vi "niGPS Direct Streaming.vi"() -> ()   [LabVIEW 2026]
doc: "This example shows how to simulate GPS signals using a real receiver location. This example also demonstrates the generation of GPS data without storing it into an intermediate binary file. The signal simulation is done based on the user input for Almanac File, Ephemeris File, Initial GPS Time of Week, Number of Frames, Receiver Location Format and Receiver Location and Receiver Velocity. The Data Creation Mode has been chosen to be Automatic. This guarantees a position fix in almost all the cases provided that the receiver location is valid and the sufficient satellites have passed the checks to be selected in simulation. \n\n\nSample ECEF values in the order of X,Y,Z in meters for different locations:\n\n\nBangalore (India) : 1.33678E+6, 6.07161E+6, 1.42381E+6 \nAustin (USA): -742817, -5.46326E+6, 3.19603E+6\nFlorence (Italy) : 4.52486E+6, 900051, 4.38947E+6 \nBrussels (Belgium) : 4.02493E+6, 304989, 4.92191E+6 \nVimercate (Italy) : 4.40941E+6, 727340, 4.53568E+6\n\nYou can find the coordinates of places easily on the web. One example is : Visit:http://www.fallingrain.com/world/"
uses:
  <vilib>/addons/Modulation/Analog/controls/Complex Data Waveform.ctl
  <vilib>/addons/Modulation/Analog/support/Validators/mod_Fractional Resample Validate.vi
  <vilib>/addons/Modulation/Analog/support/Validators/mod_Check Flush State.vi
  <vilib>/addons/Modulation/Analog/support/mod_FractionalResampler.vi
  <vilib>/addons/Modulation/Analog/support/mod_Integer Rate Interpolation.vi
  <vilib>/addons/Modulation/Analog/support/mod_Set Error Source.vi
  <vilib>/addons/Modulation/Analog/support/Validators/mod_Validate Complex Waveform.vi
  <vilib>/addons/Modulation/Analog/support/mod_PerformResampling.vi
  <vilib>/addons/Modulation/Analog/support/Validators/mod_WFErrorHandler.vi
  <instrlib>/niUSRP/niUSRP Write Tx Data (CDB Cluster).vi
  <vilib>/Utility/error.llb/Error Cluster From Error Code.vi
  <vilib>/addons/Modulation/Analog/support/mod_Resampling Factors.vi
  <vilib>/addons/Modulation/Analog/support/mod_ResamplingFilter.vi
  <vilib>/addons/Modulation/Analog/support/mod_Generate Integer Interpolation Filter.vi
  <resource>/objmgr/niGPSAttribs.rc
  <vilib>/addons/Modulation/niAMT.lvlib
panel:
  out "Waveform Graph":cluster{"t0":dbl, "dt":dbl, "Y":dbl[]}(graph)
  in  "Reference Frequency Source":string(combo)="GPS"
  in  "Stop Generation":bool
  in  "Generate GPS":bool
  in  "Freq Offset, Hz":dbl=4000000.0 format="%^.2e"
  out "coerced carrier":dbl=1575420000.0099506 format="%#_6p"
  out "coerced IQ rate":dbl=2000000.0 format="%#_6p"
  in  "device names":refnum<k15>="192.168.10.2"
  in  "IQ rate (S/s)":dbl=2000000.0 format="%#_6p"
  in  "carrier frequency":dbl=1575420000.0 format="%#_6p"
  in  "Gain":dbl format="%.2f"
  out "Consumer End":bool
  out "Producer End":bool
  out "Queue":i32(slide)=100 scale=0.0..100.0
  in  "Waveform Scaling Factor":dbl=0.5
  in  "Max Relative Power Level (dB)":dbl=10.0
  in  "Optimal Satellite Update Interval":dbl=30.0
  in  "Maximum Number of \nOptimal Satellites":i32=8
  out "Satellites Selected":string="2,5,6,7,10,12,24,30"
  out "Generation State":T1(ring)=enum."Generating Waveform"
  in  "Initial GPS Time of Week":u32=345600
  in  "Reference Power Level (dBm)":dbl=-50.0
  out "Number of Bits Created":i32(slide)=916 scale=0.0..37500.0
  out "Current GPS Time of Week":dbl=345782.82 format="%.4f"
  in  "Receiver Location":enum32{"ECEF", "LLA "}(tab)=enum."LLA "
  in  "Z":dbl=3196033.0 format="%#_f"
  in  "Y":dbl=-5463257.0 format="%#_f"
  in  "X":dbl=-742817.0 format="%#_f"
  in  "LLA":enum32{"Latitude", "Longitude", "Altitude"}(tab)
  in  "Lat.Direction":i32(ring) items=["N", "S"]
  in  "Lat.Seconds":dbl=26.3754
  in  "Lat.Minutes":dbl=50.0
  in  "Lat.Degrees":dbl=38.0
  in  "Long.Direction":i32(ring)=1 items=["E", "W"]
  in  "Long.Seconds":dbl=38.7132
  in  "Long.Minutes":dbl=2.0
  in  "Long.Degrees":dbl=105.0
  in  "Altitude":dbl=4302.0
  in  "Number of Frames":i32=25
  in  "Receiver Location Format":i32(ring)=1 items=["ECEF", "LLA"]
  in  "Ephemeris File Path":path=path "C:/Program Files (x86)/National Instruments/GPS/Ephemeris files/brdc3190.07n"
  in  "Almanac File Path":path=path "C:/Program Files (x86)/National Instruments/GPS/Almanac files/319.al3"
  out "Error Out":errorcluster
  # "NI-USRP CONFIG"
  # "GPS SETTINGS"
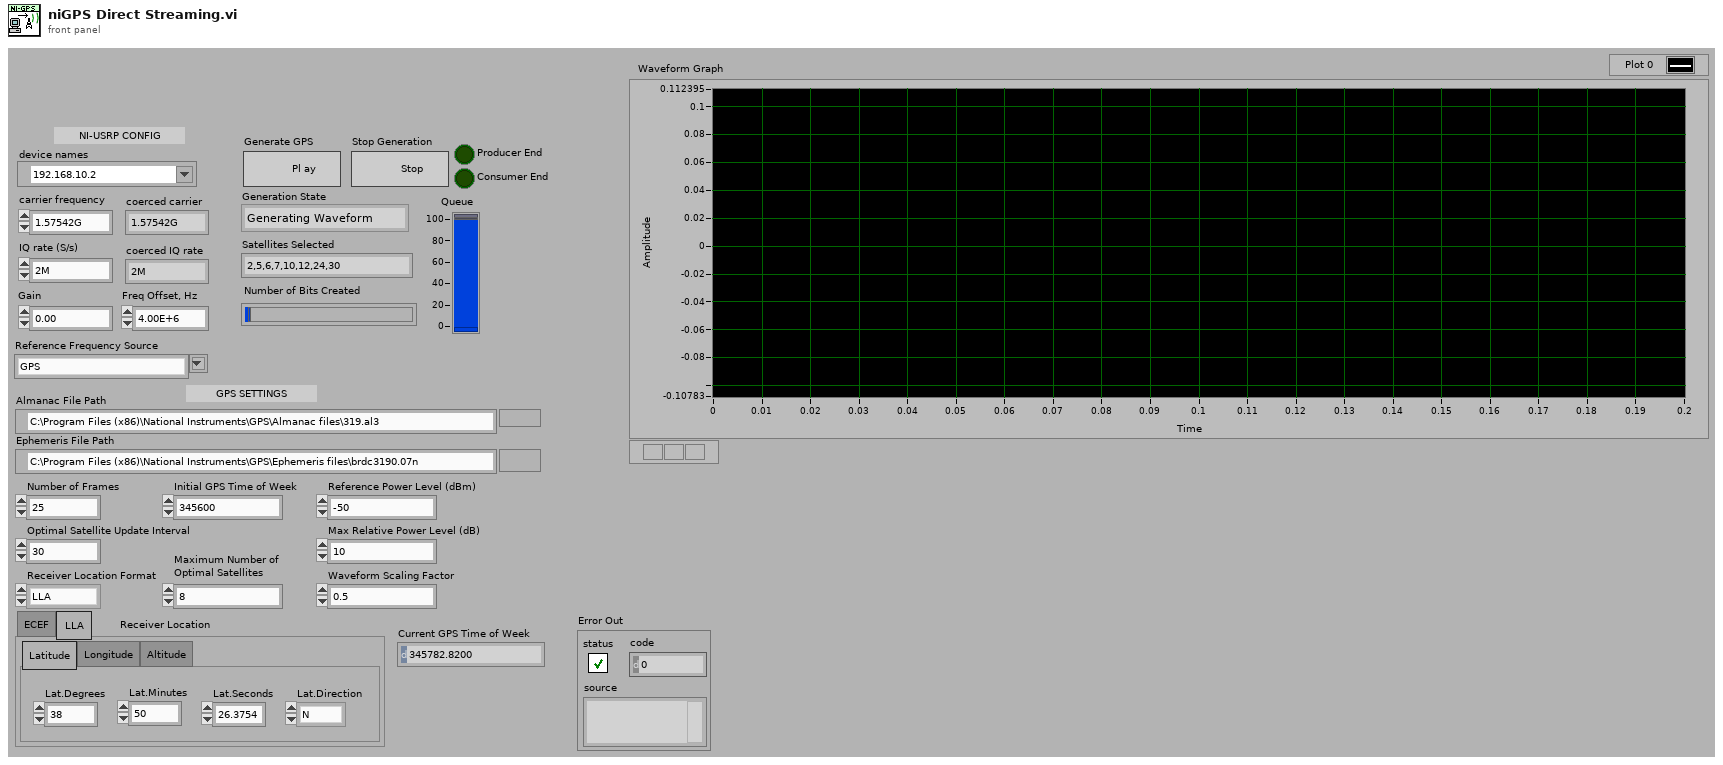
[diagram p1: front panel]
types:
  T1 = enum16{"Not Generating", "Buffering Waveform", "Generating Waveform", "Finishing Generation"}
  T2 = typedef "niAMT.lvlib/Complex Data Waveform.ctl" = cluster{"t0":dbl, "dt":dbl, "Y":cdb[]}
  T3 = typedef "gpsv1_refnum.ctl" = refnum<k20>
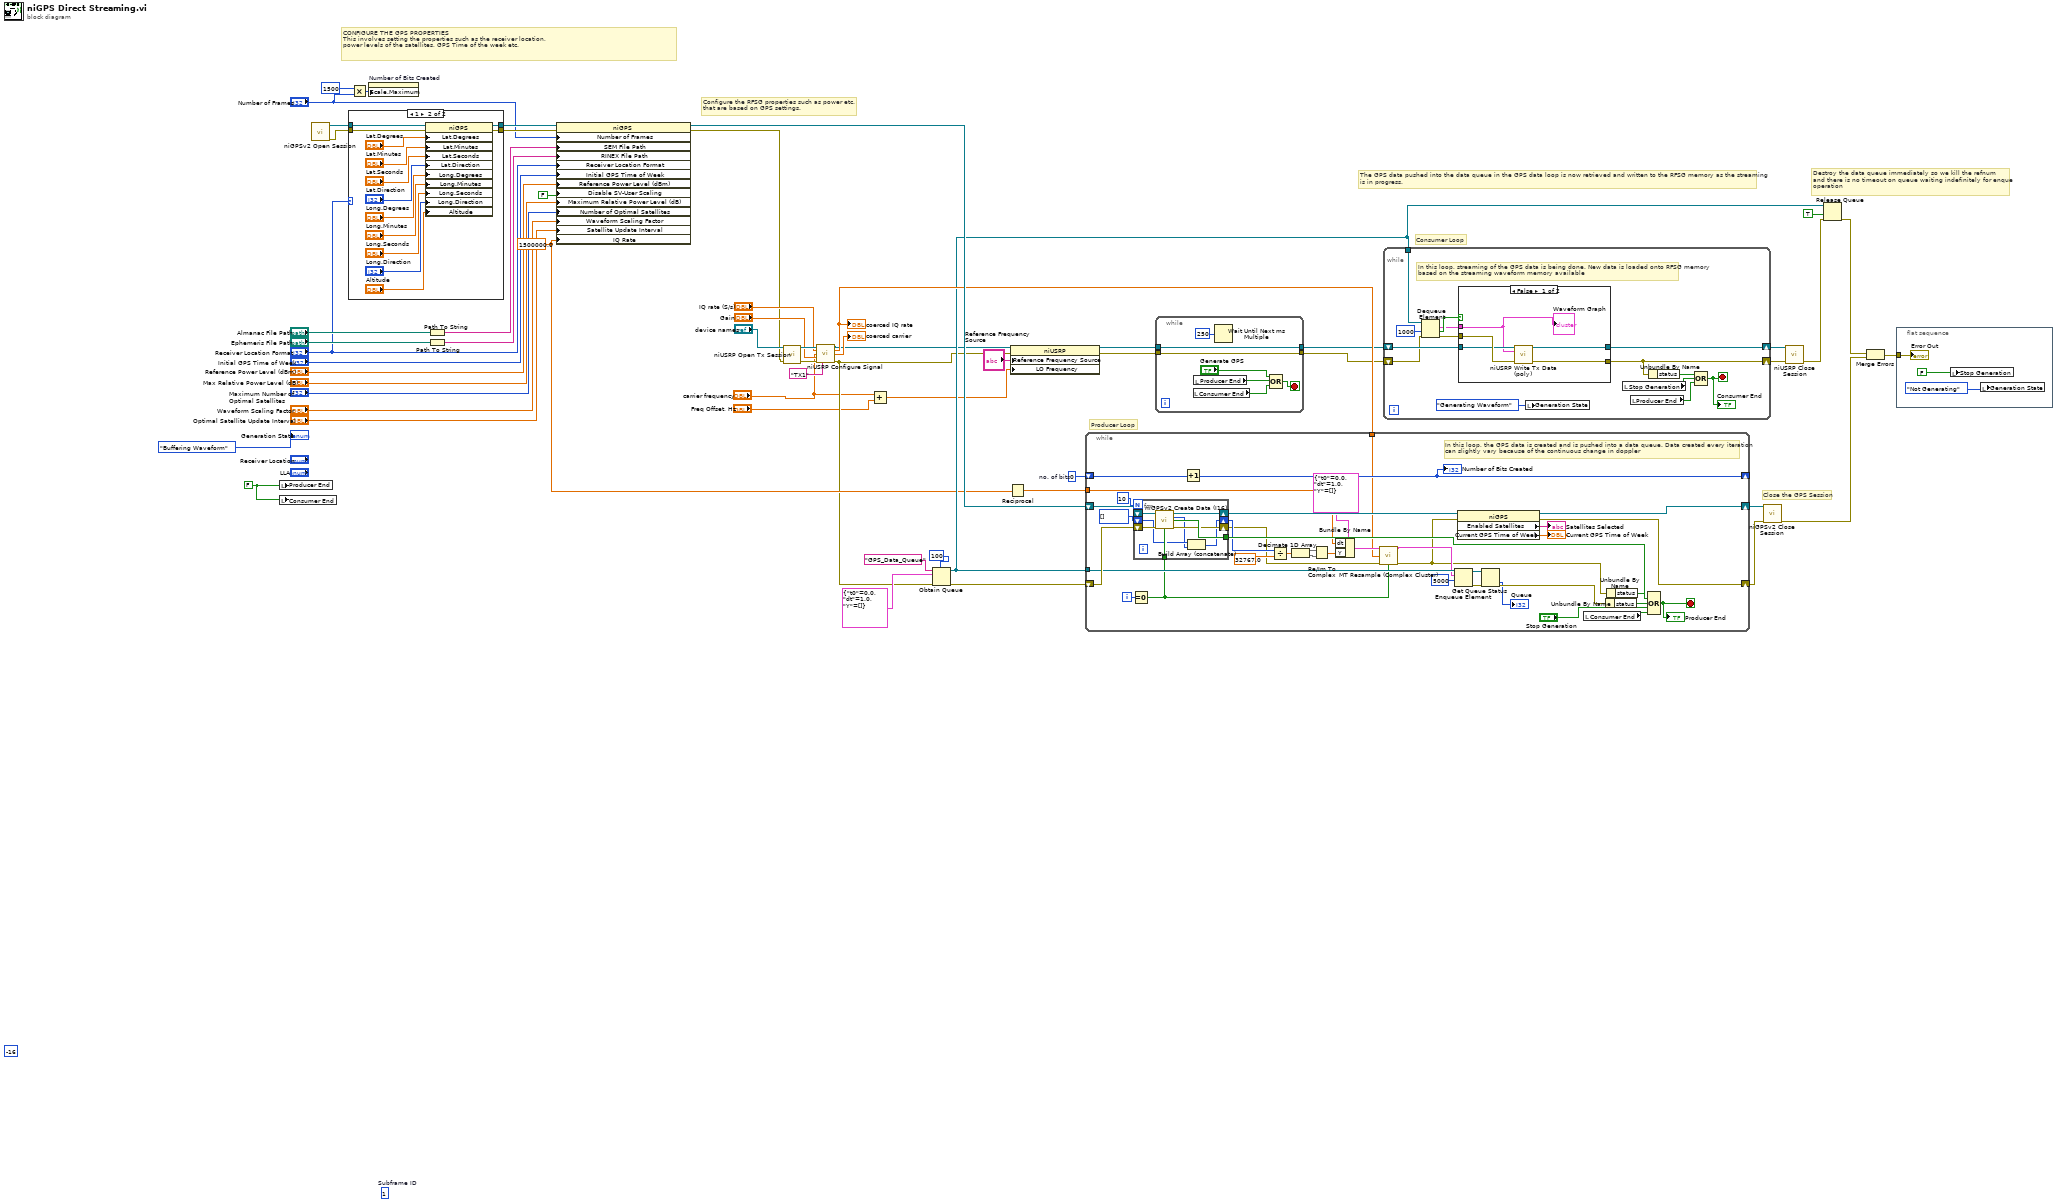
[diagram p0: block diagram]
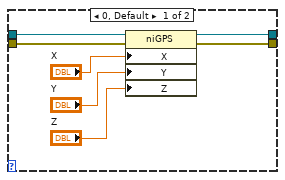
[diagram p3: hidden frame]
diagram:
  w14 = 1500000.0 ("IQ Rate")
  w31 = FALSE ("Producer End")
  w38 = 0  # no. of bits
  (unwired) i16 -16 ("n")
  (unwired) i8 1  # Subframe ID
  # "Producer Loop"
  # "Consumer Loop"
  # "The GPS data pushed into the data queue in the GPS data loop is now retrieved and written to the RFSG memory as the streaming \nis in progress."
  # "Configure the RFSG properties such as power etc. \nthat are based on GPS settings."
  # "Close the GPS Session"
  # "Destroy the data queue immediately so we kill the refnum \nand there is no timeout on queue waiting indefinitely for enque \noperation"
  # "CONFIGURE THE GPS PROPERTIES \nThis involves setting the properties such as the receiver location, \npower levels of the satellites, GPS Time of the week etc."
  n1 = local write "Producer End"(w31) -> ()
  n2 = local write "Consumer End"(w31) -> ()
  n3 = call <vilib>:"niGPSv2 Open Session.vi"() -> ("nigps session out"=w54:T3, "error out"=w34:errorcluster)  [unwired: 14 in]
  n4 = case shown="1" "Receiver Location Format" {
    tunnel: w54 -> [w65 w77]
    tunnel: w34 -> [w63 w76]
    tunnel: [w64 w78] -> w45
    tunnel: [w62 w75] -> w53
    frame 0, Default {
      n5 = property class="niGPS"(reference=w65, error in=w63, "X"="X", "Y"="Y", "Z"="Z") -> (reference out=w64:T3, error out=w62:errorcluster)
    }
    frame 1 {
      n6 = property class="niGPS"(reference=w77, error in=w76, "Lat.Degrees"="Lat.Degrees", "Lat.Minutes"="Lat.Minutes", "Lat.Seconds"="Lat.Seconds", "Lat.Direction"="Lat.Direction", "Long.Degrees"="Long.Degrees", "Long.Minutes"="Long.Minutes", "Long.Seconds"="Long.Seconds", "Long.Direction"="Long.Direction", "Altitude"="Altitude") -> (reference out=w78:T3, error out=w75:errorcluster)
    }
  }
  n7 = Multiply(x=1500, y="Number of Frames") -> (x*y=w51:i32)
  n8 = property on="Number of Bits Created" class="Slide (strict)"("Scale.Maximum"=w51) -> ()  [unwired: 2 in, 2 out]
  n9 = Path To String(path="Almanac File Path") -> (string=w55:string)
  n10 = Path To String(path="Ephemeris File Path") -> (string=w58:string)
  n11 = property class="niGPS"(reference=w45, error in=w53, "Number of Frames"="Number of Frames", "SEM File Path"=w55, "RINEX File Path"=w58, "Receiver Location Format"="Receiver Location Format", "Initial GPS Time of Week"="Initial GPS Time of Week", "Reference Power Level (dBm)"="Reference Power Level (dBm)", "Disable SV-User Scaling"=FALSE, "Maximum Relative Power Level (dB)"="Max Relative Power Level (dB)", "Number of Optimal Satellites"="Maximum Number of \nOptimal Satellites", "Waveform Scaling Factor"="Waveform Scaling Factor", "Satellite Update Interval"="Optimal Satellite Update Interval", "IQ Rate"=w14) -> (reference out=w30:T3, error out=w10:errorcluster)
  n12 = call <instrlib>:"niUSRP Open Tx Session.vi"("device names"="device names", "error in (no error)"=w10) -> ("session handle out"=w29:refnum<k15>, "error out"=w9:errorcluster)  [unwired: 12 in]
  n13 = call <instrlib>:"niUSRP Configure Signal.vi"("session handle"=w29, "IQ rate"="IQ rate (S/s)", "carrier frequency"="carrier frequency", "gain"="Gain", "error in (no error)"=w9, "active antenna"="TX1") -> ("session handle out"=w13:refnum<k15>, "coerced IQ rate"=w17:dbl, "coerced carrier frequency"=→"coerced carrier":dbl, "error out"=w11:errorcluster)  [unwired: 5 in, 1 out]
  "coerced IQ rate" <- w17
  n14 = Add(x="carrier frequency", y="Freq Offset, Hz") -> (x+y=w1:dbl)
  n15 = Obtain Queue(max queue size (-1, unlimited)=100, name (unnamed)="GPS_Data_Queue", element data type=T2 {"t0"=0.0, "dt"=1.0, "Y"=[]} ("input complex waveform"), error in (no error)=w11) -> (queue out=w16:refnum<queue>, error out=w36:errorcluster)  [unwired: 1 in, 1 out]
  n16 = Reciprocal(x=w14) -> (1/x=w19:dbl)
  n17 = property class="niUSRP"(reference=w13, error in=w11, "Reference Frequency Source"="Reference Frequency Source", "LO Frequency"=w1) -> (reference out=w8:refnum<k15>, error out=w7:errorcluster)
  n18 = while {
    shift-right: [w110] -> w32
    shift-left: w36 -> [w115]
    shift-right: [w111] -> w39
    shift-left: w30 -> [w116]
    shift-right: [w105] -> _
    shift-left: w38 -> [w106]
    tunnel: w19 -> [w84]
    tunnel: w17 -> [w90]
    tunnel: w16 -> [w86]
    i -> [w114]
    stop <- w85 stop-if-true
    # "In this loop, the GPS data is created and is pushed into a data queue. Data created every iteration\ncan slightly vary because of the continuous change in doppler"
    n19 = Equal To 0?(x=w114) -> (x = 0?=w82:bool)
    n20 = for {
      N: 10 -> [_]
      tunnel: w82 -> [w123]
      tunnel: [w121] -> w109
      shift-right: [w122] -> w112
      shift-left: w116 -> [w125]
      shift-right: [w117] -> w92
      shift-left: i16[] [] ("gps waveform") -> [w119]
      shift-right: [w120] -> w88
      shift-left: w115 -> [w124]
      n21 = call <vilib>:"niGPSv2 Create Data (I16).vi"("nigps session"=w125, "error in"=w124, "reset?"=w123) -> ("nigps session out"=w122:T3, "gps waveform"=w118:i16[], "done?"=w121:bool, "error out"=w120:errorcluster)  [unwired: 9 in]
      n22 = Build Array (concatenate)(w119, w118) -> (w117:i16[])
    }
    n23 = Increment(x=w106) -> (x+1=w105:i32)
    "Number of Bits Created" <- w105
    n24 = Divide(x=w92, y=32767.0 ("n")) -> (x/y=w89:dbl[])
    n25 = Decimate 1D Array(w89) -> (w93:dbl[], w94:dbl[])
    n26 = Re/Im To Complex(1:w94, 2:w93) -> (0:w83:cdb[])
    n27 = Bundle By Name(cluster=T2 {"t0"=0.0, "dt"=1.0, "Y"=[]} ("input complex waveform"), "dt"=w84, "Y"=w83) -> (w96:T2)
    n28 = call <vilib>:"MT Resample (Complex Cluster).vi"("input complex waveform"=w96, "desired sample rate (Hz)"=w90, "error in (no error)"=w88, "reset? (T)"=w82) -> ("output complex waveform"=w80:T2, "error out"=w79:errorcluster)  [unwired: 10 in]
    n29 = Enqueue Element(queue=w86, element=w80, timeout in ms (-1)=5000) -> (queue out=w104:refnum<queue>, error out=w103:errorcluster)  [unwired: 1 in, 1 out]
    n30 = property class="niGPS"(reference=w112, error in=w79) -> (reference out=w111:T3, error out=w110:errorcluster, "Enabled Satellites"=→"Satellites Selected":string, "Current GPS Time of Week"=→"Current GPS Time of Week":dbl)
    n31 = Get Queue Status(queue=w104, error in (no error)=w103) -> (error out=w102:errorcluster, # elements in queue=→"Queue":i32)  [unwired: 1 in, 6 out]
    n32 = local read "Consumer End"() -> (w101:bool)
    n33 = Unbundle By Name(w102) -> ("status"=w113:bool)
    n34 = Unbundle By Name(w79) -> ("status"=w99:bool)
    n35 = Compound Arithmetic op=OR(w99, w109, w113, "Stop Generation", w101) -> (w85:bool)
    "Producer End" <- w85
  }
  n36 = while {
    tunnel: w8 -> [w132]
    tunnel: w7 -> [w131]
    tunnel: [w132] -> w6
    tunnel: [w131] -> w5
    stop <- w129 stop-if-true
    n37 = local read "Consumer End"() -> (w126:bool)
    n38 = local read "Producer End"() -> (w127:bool)
    n39 = Wait Until Next ms Multiple(millisecond multiple=u32 250) -> ()  [unwired: 1 out]
    n40 = Compound Arithmetic op=OR("Generate GPS", w127, w126) -> (w129:bool)
  }
  n41 = while {
    shift-right: [w146] -> w23
    shift-left: w6 -> [w141]
    shift-right: [w145] -> w24
    shift-left: w5 -> [w136]
    tunnel: w16 -> [w134]
    stop <- w133 stop-if-true
    # "In this loop, streaming of the GPS data is being done. New data is loaded onto RFSG memory \nbased on the streaming waveform memory available"
    n42 = Dequeue Element(queue=w134, timeout in ms (-1)=1000, error in (no error)=w136) -> (element=w135:T2, timed out?=w138:bool, error out=w137:errorcluster)  [unwired: 1 out]
    n43 = case shown="False" w138 {
      tunnel: w141 -> [w148 w153]
      tunnel: [w150 w152] -> w145
      tunnel: [w151 w153] -> w146
      tunnel: w137 -> [w149 w152]
      tunnel: w135 -> [w147 _]
      frame False {
        n44 = call-poly <instrlib>:"niUSRP Write Tx Data (poly).vi"("session handle"=w148, "data"=w147, "error in (no error)"=w149) -> ("session handle out"=w151:refnum<k15>, "error out"=w150:errorcluster)  [unwired: 11 in]
        "Waveform Graph" <- w147
      }
      frame True {
      }
    }
    n45 = local write "Generation State"(T1."Generating Waveform" ("Generation State")) -> ()
    n46 = local read "Stop Generation"() -> (w143:bool)
    n47 = local read "Producer End"() -> (w142:bool)
    n48 = Unbundle By Name(w145) -> ("status"=w144:bool)
    n49 = Compound Arithmetic op=OR(w144, w143, w142) -> (w133:bool)
    "Consumer End" <- w133
  }
  n50 = call <vilib>:"niGPSv2 Close Session.vi"("nigps session"=w39, "error in"=w32) -> ("error out"=w35:errorcluster)  [unwired: 13 in]
  n51 = call <instrlib>:"niUSRP Close Session.vi"("session handle"=w23, "error in (no error)"=w24) -> ("error out"=w22:errorcluster)  [unwired: 13 in]
  n52 = Release Queue(queue=w16, force destroy? (F)=TRUE, error in (no error)=w22) -> (error out=w21:errorcluster)  [unwired: 2 out]
  n53 = Merge Errors(w21, w35) -> (w33:errorcluster)
  n54 = flat-sequence {
    tunnel: w33 -> [w154]
    frame #0 {
      n55 = local write "Stop Generation"(FALSE ("Stop")) -> ()
      n56 = local write "Generation State"(T1."Not Generating" ("Generation State")) -> ()
      "Error Out" <- w154
    }
  }
  "Generation State" <- T1."Buffering Waveform" ("Generation State")
